vi "Read.vi"(6 "prioritize Cache? (F)":bool, 7 "Qualified Name":string, 8 "error in (no error)":errorcluster, 9 "Default Values":variant[](array[variant]), 10 "keys in":string[](array[string]), 11 "ConfigManager in":refnum<class "ConfigManager.lvclass">) -> (0 "error out":errorcluster, 1 "Values":variant[](array[variant]), 2 "keys":string[](array[string]), 3 "ConfigManager out":refnum<class "ConfigManager.lvclass">, 4 "All Found?":bool, 5 "Any Found?":bool)   [LabVIEW 2013, in "CfgManager.lvlib" / "ConfigManager.lvclass"]
uses:
  ConfigManager.lvclass
  ConfigManager.lvclass/ConfigManager.ctl
  Encoding/Encoding.lvclass
  Encryption/Encryption.lvclass
  <vilib>/LabVIEW Open Source Project/Serializer/Serializer/Serializer.lvclass
  <vilib>/LabVIEW Open Source Project/Serializer/Serializer.PlainText/Serializer.PlainText.lvclass
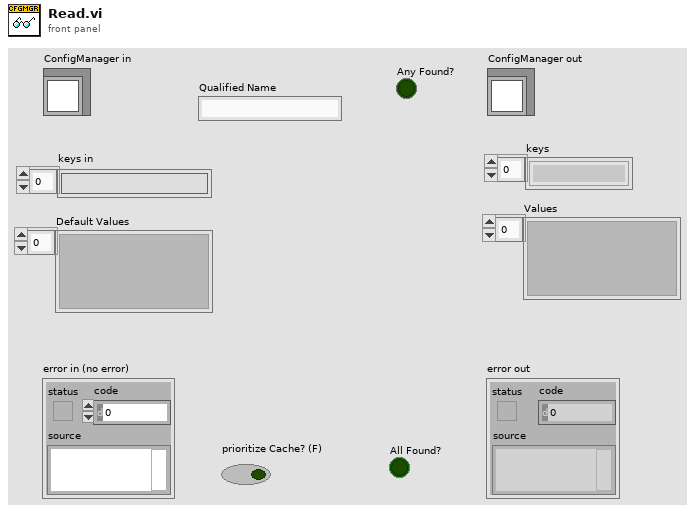
[diagram p1: front panel]
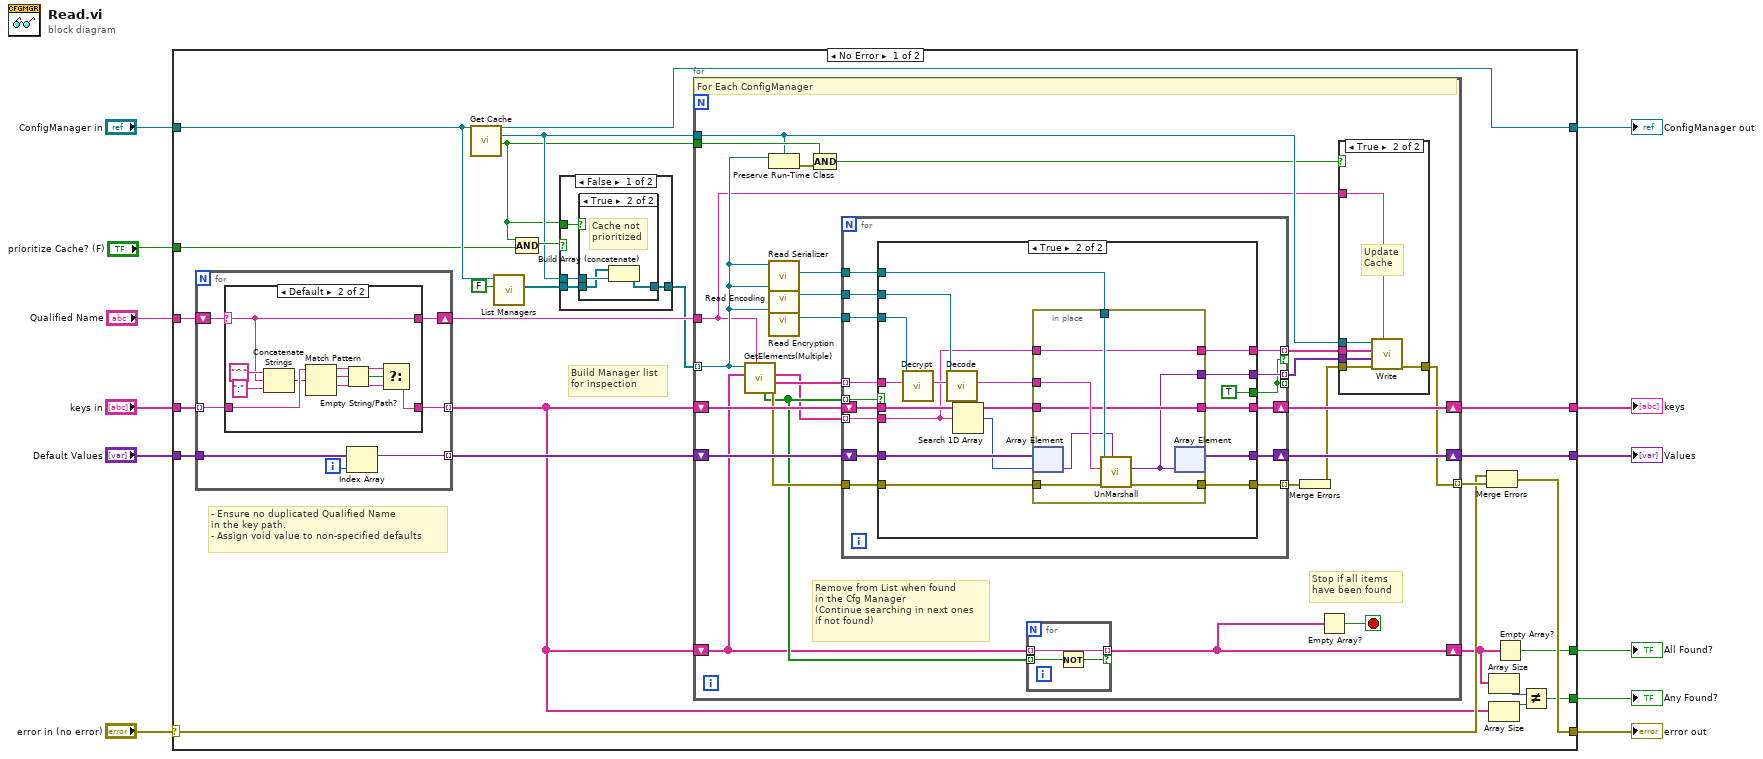
[diagram p0: block diagram]
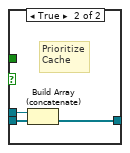
[diagram p3: hidden frame]
diagram:
  n1 = case shown="No Error" "error in (no error)" {
    selector: "error in (no error)" -> [w32 w149]
    tunnel: [w31 w149] -> w11
    tunnel: [w19 w148] -> w9
    tunnel: "ConfigManager in" -> [w26 w148]
    tunnel: "keys in" -> [w30 w146]
    tunnel: "Default Values" -> [w36 w147]
    tunnel: [w35 w147] -> w6
    tunnel: [w34 w146] -> w5
    tunnel: "Qualified Name" -> [w29 _]
    tunnel: "prioritize Cache? (F)" -> [w22 _]
    tunnel: [w18 _] -> w2
    tunnel: [w13 _] -> w1
    frame No Error {
      # "Build Manager list\nfor inspection"
      # "- Ensure no duplicated Qualified Name\nin the key path.\n- Assign void value to non-specified defaults"
      n2 = for {
        tunnel: w36 -> [w54]
        tunnel: [w53] -> w37 mode=indexing
        tunnel: w30 -> [w52] mode=indexing
        tunnel: [w49] -> w16 mode=indexing
        shift-right: [w50] -> w28
        shift-left: w29 -> [w51]
        i -> [w55]
        n3 = case shown="Default" w51 {
          selector: w51 -> [w57 w64]
          tunnel: w52 -> [w56 w67]
          tunnel: [w57 w64] -> w50
          tunnel: [w56 w58] -> w49
          frame "" {
          }
          frame Default {
            n4 = Concatenate Strings("^" ("string"), w64, ":" ("string")) -> (w66:string)
            n5 = Match Pattern(string=w67, regular expression=w66) -> (before substring=w61:string, match substring=w63:string, after substring=w60:string)  [unwired: 1 in, 1 out]
            n6 = Empty String/Path?(string/path=w63) -> (empty?=w62:bool)
            n7 = Select(t=w61, s=w62, f=w60) -> (s? t:f=w58:string)
          }
        }
        n8 = Index Array(array=w54, index=w55) -> (element=w53:variant)
      }
      n9 = call-dynamic "Get Cache.vi"("ConfigManager in"=w26) -> ("found?"=w20:bool, "Cache"=w21:refnum<class "ConfigManager.Cache.lvclass">, "ConfigManager out"=w19:refnum<class "ConfigManager.lvclass">)  [unwired: 8 in]
      n10 = call-dynamic "List Managers.vi"("Include Cache? (F)"=FALSE, "ConfigManager in"=w26) -> ("List"=w25:refnum<class "ConfigManager.lvclass">[])  [unwired: 8 in, 1 out]
      n11 = Compound Arithmetic op=AND(w20, w22) -> (w23:bool)
      n12 = case shown="False" w23 {
        tunnel: w21 -> [w40 w48]
        tunnel: w25 -> [w39 w47]
        tunnel: [w38 w46] -> w24
        tunnel: w20 -> [w41 _]
        frame False {
          n13 = case shown="True" w41 {
            tunnel: w40 -> [_ w45]
            tunnel: w39 -> [w42 w44]
            tunnel: [w42 w43] -> w38
            frame False {
              # "No cache\nfound"
            }
            frame True {
              # "Cache not\nprioritized"
              n14 = Build Array (concatenate)(w44, w45) -> (w43:refnum<class "ConfigManager.lvclass">[])
            }
          }
        }
        frame True {
          # "Prioritize\nCache"
          n15 = Build Array (concatenate)(w48, w47) -> (w46:refnum<class "ConfigManager.lvclass">[])
        }
      }
      n16 = for {
        tunnel: w24 -> [w84] mode=indexing
        shift-right: [w72] -> w17
        shift-left: w16 -> [w69]
        shift-right: [w89] -> w35
        shift-left: w37 -> [w92]
        shift-right: [w90] -> w34
        shift-left: w16 -> [w91]
        tunnel: [w78] -> w33 mode=indexing
        tunnel: w28 -> [w76]
        tunnel: w21 -> [w81]
        tunnel: w20 -> [w82]
        stop <- w73 stop-if-true
        # "Remove from List when found\nin the Cfg Manager\n(Continue searching in next ones\nif not found)"
        # "Stop if all items\nhave been found"
        # "For Each ConfigManager"
        n17 = call-dynamic "GetElements(Multiple).vi"("Qualified Name"=w76, "keys"=w69, "ConfigManager in"=w84) -> ("error out"=w74:errorcluster, "Values"=w70:string[], "Keys"=w68:string[], "Found"=w71:bool[])  [unwired: 4 in, 1 out]
        n18 = Preserve Run-Time Class(object in=w84, 2:w81) -> (error out=w83:errorcluster)  [unwired: 1 in, 1 out]
        n19 = call "Read Serializer.vi"("ConfigManager in"=w84) -> ("Serializer"=w87:refnum<class "Serializer.lvclass">)  [unwired: 9 in, 1 out]
        n20 = call "Read Encoding.vi"("ConfigManager in"=w84) -> ("Encoding"=w88:refnum<class "Encoding.lvclass">)  [unwired: 9 in, 1 out]
        n21 = call "Read Encryption.vi"("ConfigManager in"=w84) -> ("Encryption"=w85:refnum<class "Encryption.lvclass">)  [unwired: 9 in, 1 out]
        n22 = Compound Arithmetic op=AND(w82, w83) -> (w75:bool)
        n23 = for {
          tunnel: w70 -> [w117] mode=indexing
          tunnel: w87 -> [w116]
          tunnel: w88 -> [w115]
          tunnel: w71 -> [w114] mode=indexing
          shift-right: [w111] -> w90
          shift-left: w91 -> [w113]
          shift-right: [w110] -> w89
          shift-left: w92 -> [w112]
          tunnel: w74 -> [w109]
          tunnel: [w108] -> w86 mode=indexing
          tunnel: w68 -> [w107] mode=indexing
          tunnel: w85 -> [w106]
          tunnel: [w105] -> w79 mode=indexing if=w103
          tunnel: [w104] -> w80 mode=indexing if=w103
          tunnel: [w103] -> _ mode=indexing
          n24 = case shown="True" w114 {
            tunnel: w117 -> [_ w127]
            tunnel: w116 -> [_ w133]
            tunnel: w115 -> [_ w137]
            tunnel: w113 -> [w120 w130]
            tunnel: w112 -> [w119 w136]
            tunnel: [w120 w131] -> w111
            tunnel: [w119 w135] -> w110
            tunnel: w109 -> [w118 w129]
            tunnel: [w118 w128] -> w108
            tunnel: w107 -> [_ w122]
            tunnel: w106 -> [_ w125]
            tunnel: [_ w124] -> w105
            tunnel: [_ w123] -> w104
            tunnel: [_ TRUE] -> w103
            frame False {
            }
            frame True {
              n25 = call-dynamic "Decrypt.vi"("Encrypted String"=w127, "Encryption in"=w125) -> ("String"=w126:string)  [unwired: 8 in, 1 out]
              n26 = call-dynamic "Decode.vi"("Encoded String"=w126, "CfgEncoding in"=w137) -> ("String"=w132:string)  [unwired: 8 in, 1 out]
              n27 = Search 1D Array(1D array=w130, element=w122) -> (index of element=w134:i32)  [unwired: 1 in]
              n28 = in-place {
                in-place-border: w133 -> [w145]
                in-place-border: w132 -> [w144]
                in-place-border: [w142] -> w131
                in-place-border: w130 -> [w142]
                in-place-border: w129 -> [w141]
                in-place-border: [w140] -> w128
                in-place-border: [w139] -> w124
                in-place-border: [w138] -> w123
                in-place-border: w122 -> [w138]
                n29 = in-place-array #1(w136, w134) -> (w143:variant)
                n30 = call <vilib>:"UnMarshall.vi"("Type"=w143, "error in (no error)"=w141, "String"=w144, "Serializer in"=w145) -> ("error out"=w140:errorcluster, "Variant"=w139:variant)  [unwired: 5 in, 1 out]
                n31 = in-place-array #1(w139) -> (w135:variant[])  [unwired: 1 out]
              }
            }
          }
        }
        n32 = for {
          tunnel: w69 -> [w102] mode=indexing
          tunnel: w71 -> [w101] mode=indexing
          tunnel: [w102] -> w72 mode=indexing if=w100
          n33 = Not(x=w101) -> (.not. x?=w100:bool)
        }
        n34 = Merge Errors(w86) -> (w77:errorcluster)
        n35 = Empty Array?(array=w72) -> (empty?=w73:bool)
        n36 = case shown="True" w75 {
          tunnel: w81 -> [_ w99]
          tunnel: w80 -> [_ w98]
          tunnel: w79 -> [_ w97]
          tunnel: [w93 w94] -> w78
          tunnel: w77 -> [w93 w96]
          tunnel: w76 -> [_ w95]
          frame False {
          }
          frame True {
            # "Update\nCache"
            n37 = call "Write.vi"("Qualified Name"=w95, "error in (no error)"=w96, "Values"=w97, "keys"=w98, "ConfigManager in"=w99) -> ("error out"=w94:errorcluster)  [unwired: 4 in, 2 out]
          }
        }
      }
      n38 = Merge Errors(w32, w33) -> (w31:errorcluster)
      n39 = Array Size(array=w17) -> (size(s)=w14:i32)
      n40 = Array Size(array=w16) -> (size(s)=w15:i32)
      n41 = Empty Array?(array=w17) -> (empty?=w18:bool)
      n42 = Not Equal?(x=w14, y=w15) -> (x != y?=w13:bool)
    }
    frame Error {
    }
  }
  "error out" <- w11
  "ConfigManager out" <- w9
  "Values" <- w6
  "keys" <- w5
  "All Found?" <- w2
  "Any Found?" <- w1
